vi "Host_ErrOnly.vi"(11 "error in":errorcluster) -> (3 "error out":errorcluster)   [LabVIEW 2018]
doc: "Use this template to build a VI to use as a subVI."
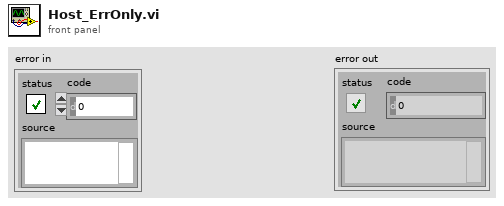
[diagram p1: front panel]
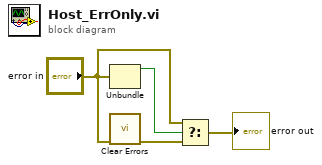
[diagram p0: block diagram]
diagram:
  n1 = Unbundle("error in") -> ("status"=w3:bool)  [unwired: 2 out]
  n2 = call <vilib>:"Clear Errors.vi"("error in (no error)"="error in") -> ("error out"=w2:errorcluster)  [unwired: 5 in, 1 out]
  n3 = Select(t="error in", s=w3, f=w2) -> (s? t:f=→"error out":errorcluster)
